vi "Set_MultiVar_Values.vi"(8 "error in (no error)":errorcluster, 9 "varValues":dbl[](array[numeric]) format="%#_13g", 10 "varNames":string[](array[string]), 11 "muExpr in":refnum<class "mupExpr.lvclass">) -> (0 "error out":errorcluster, 3 "muExpr out":refnum<class "mupExpr.lvclass">)   [LabVIEW 2015, in "mupExpr.lvclass"]
doc: "Set the values of a list of variables.\n\nIf any variable is not found, a warning is generated."
uses:
  mupExpr.lvclass
  mupExpr.lvclass/mupExpr.ctl
  mupLib/mupSetVarValue.vi
  <vilib>/Utility/error.llb/Error Cluster From Error Code.vi
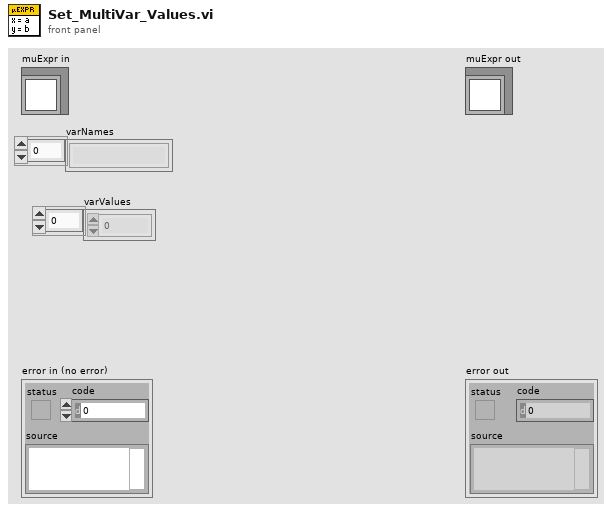
[diagram p1: front panel]
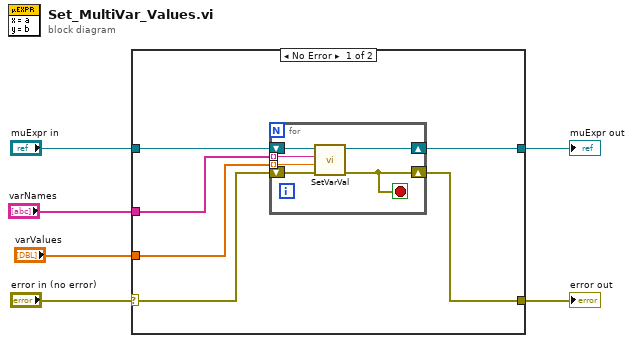
[diagram p0: block diagram]
diagram:
  n1 = case shown="No Error" "error in (no error)" {
    selector: "error in (no error)" -> [w8 w19]
    tunnel: "varValues" -> [w12 _]
    tunnel: "varNames" -> [w11 _]
    tunnel: "muExpr in" -> [w10 w20]
    tunnel: [w7 w19] -> w3
    tunnel: [w9 w20] -> w2
    frame No Error {
      n2 = for {
        tunnel: w11 -> [w18] mode=indexing
        tunnel: w12 -> [w17] mode=indexing
        shift-right: [w13] -> w7
        shift-left: w8 -> [w16]
        shift-right: [w14] -> w9
        shift-left: w10 -> [w15]
        stop <- w13 stop-if-true
        n3 = call "SetVarVal.vi"("error in (no error)"=w16, "varValue"=w17, "varName"=w18, "muExpr in"=w15) -> ("error out"=w13:errorcluster, "muExpr out"=w14:refnum<class "mupExpr.lvclass">)  [unwired: 6 in]
      }
    }
    frame Error {
    }
  }
  "error out" <- w3
  "muExpr out" <- w2
